vi "Advanced SCP File Download.vi"() -> ()   [LabVIEW 2018]
doc: "Downloads, or receives, any file from a remote SSH server in an efficient, iterative manner. This is similar to the SCP command line utility when transferring, or copying, a remote file to a local destination. Provides advanced functionality to monitoring and optimize performance."
uses:
  Toolkit/Session/Support/Create from SSH.vi
  Toolkit/Session/Support/Password Authentication.vi
  Toolkit/Channel/Support/Create from SCP Receive.vi
  Toolkit/Channel/Support/Destroy to Session.vi
  Toolkit/Session/Support/Destroy to SSH.vi
  Toolkit/SSH/SSH.lvclass
  Toolkit/Session/Session.lvclass
  Toolkit/Channel/Channel.lvclass
panel:
  in  "Abort Download":bool
  out "Download Progress":dbl(slide) scale=0.0..1.0
  out "Bytes Downloaded":u64
  out "Block Download Rate":dbl format="%.3p"
  out "File Download Rate":dbl format="%.3p"
  out "File Download Time":dbl format="%<%H:%M:%S%3u>t"
  in  "Block Size":u64=30000 max=30000
  in  "Remote File":string
  in  "Local File":path
  in  "Remote SSH Server":string
  in  "Password":string
  in  "Username":string
  # "Overview: Demonstrates transferring, or downloading, a remote file from a SSH server, similar to the SCP command line utility with advanced functionality\nInstructions:\n1. Enter the IP address or host name of the remote SSH server. This can be a CompactRIO (cRIO) running the National Instruments Linux Real-Time (NI Linux RT) operating system with the Enable Secure Shell Server (sshd) checkbox checked. \n2. Enter a username. If using a cRIO with a default configuration, then the username is \"admin\".\n3. Enter a password for the username. If using a cRIO with a default configuration, then the password is blank (empty).\n4. Enter the path and/or filename of the remote file to download. Typically, this is a POSIX/UNIX file path with a backslash, \"/\", use to separate directories and the default directory is the remote user's home directory, i.e. \"/home/admin\" on a default configured cRIO.\n5. Select a destination on the local computer for the transfer/download from the remote SSH server.\n6. Run this VI."
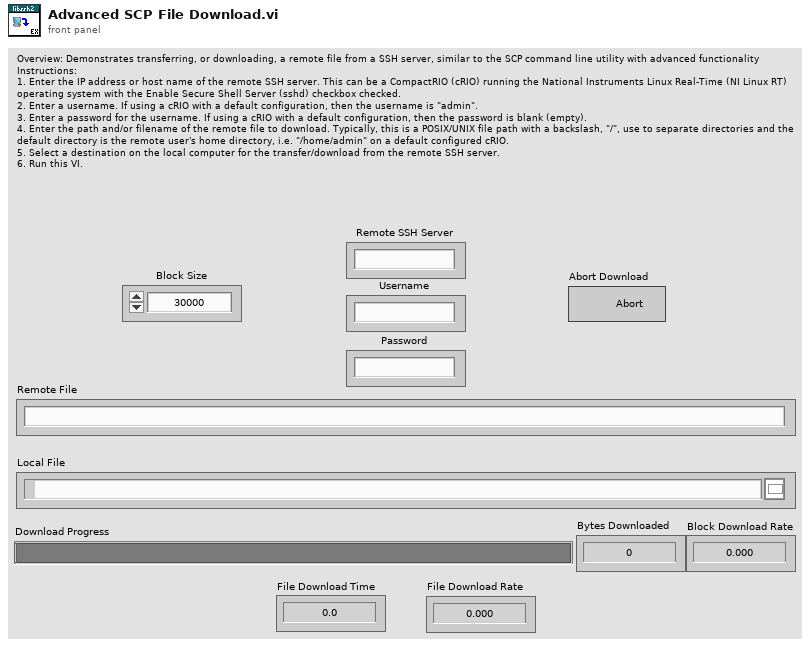
[diagram p1: front panel]
types:
  T1 = enum16{"open", "replace", "create", "open or create", "replace or create", "replace or create with confirmation"}
  T2 = typedef "Toolkit.lvlib/Permissions.ctl" = cluster{"Owner":T3, "Group":T3, "Others":T3}
  T3 = typedef "Toolkit.lvlib/Modes.ctl" = cluster{"Read":bool, "Write":bool, "Execute":bool}
  T4 = cluster{"Access Time":u64, "File Size":u64, "Modified Time":u64, "Permissions":T2}
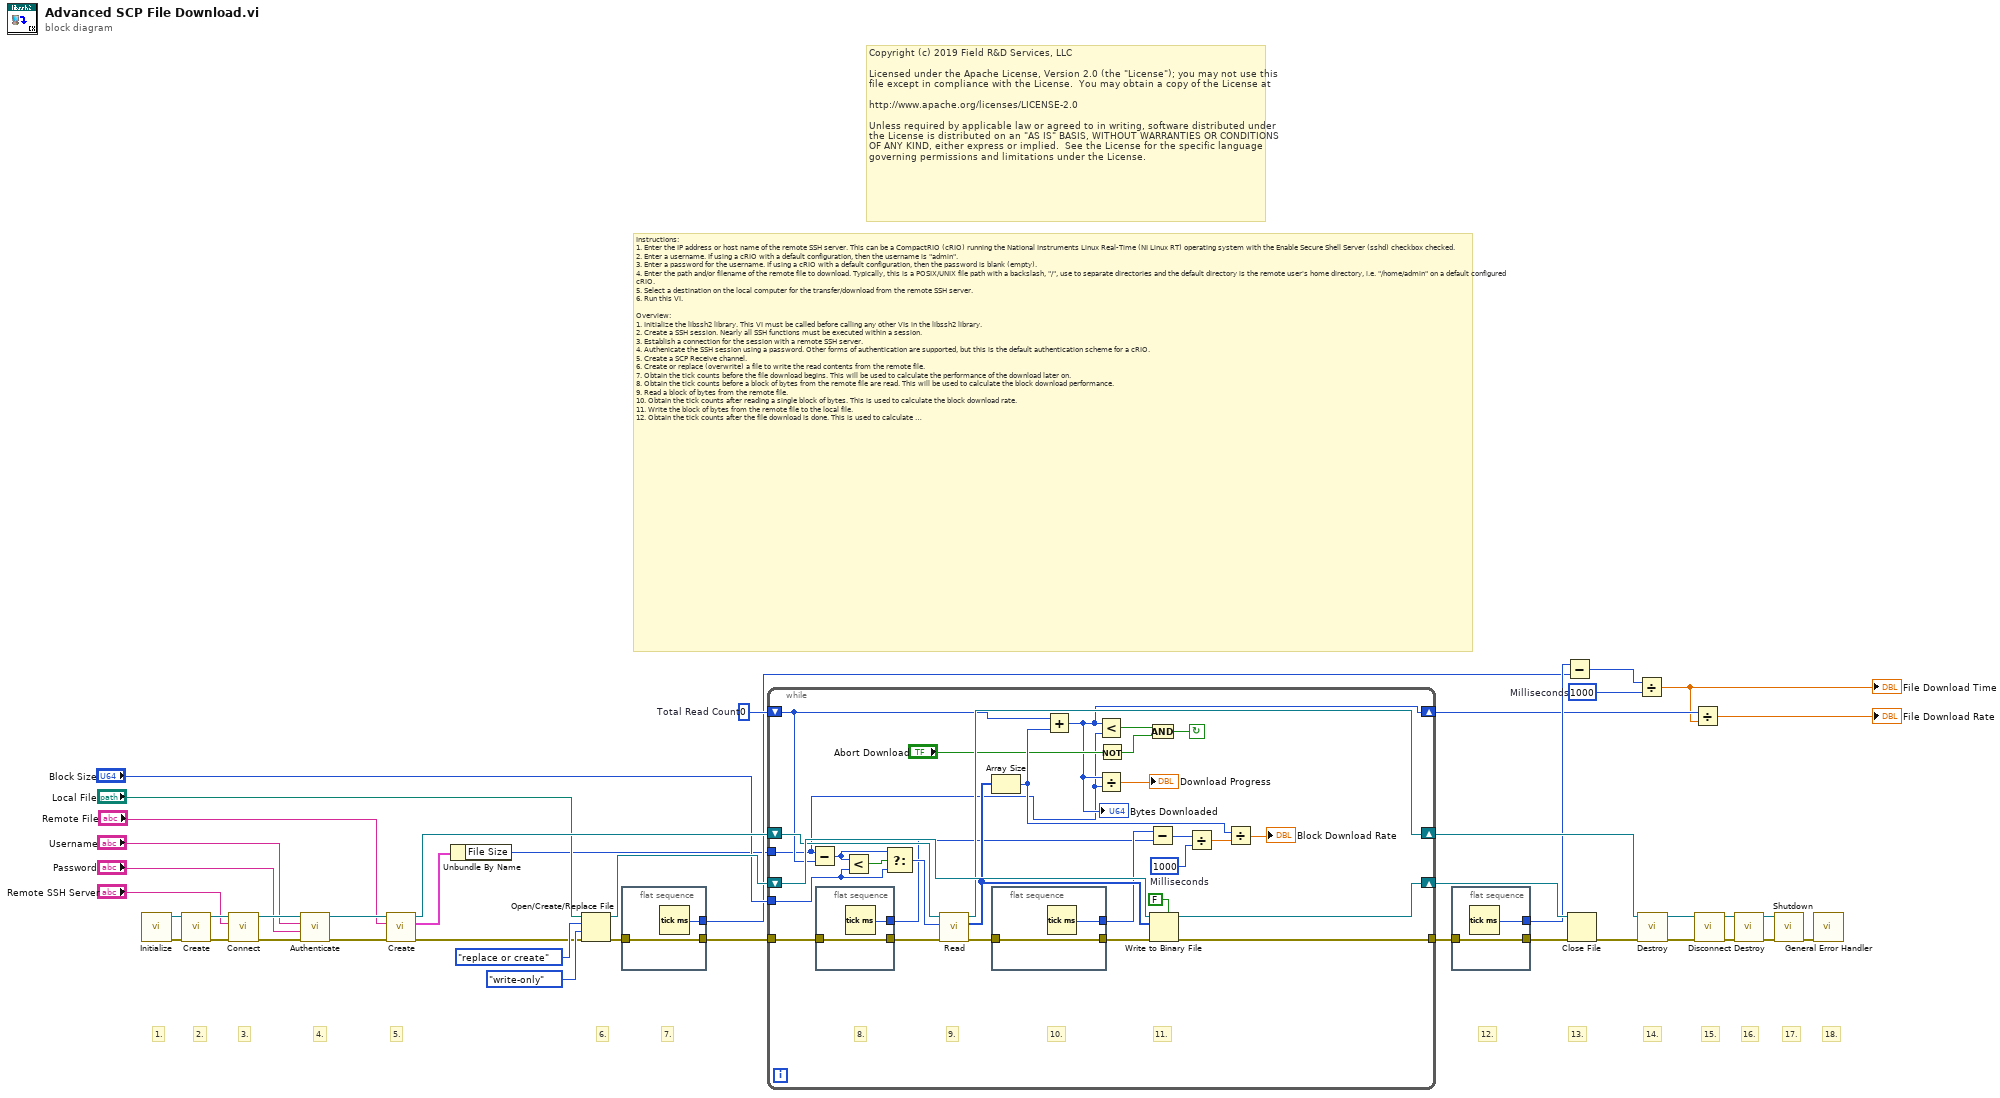
[diagram p0: block diagram]
diagram:
  w10 = u32 1000  # Milliseconds
  w19 = u64 0  # Total Read Count
  # "Copyright (c) 2019 Field R&D Services, LLC\n\nLicensed under the Apache License, Version 2.0 (the \"License\"); you may not use this file except in compliance with the License.  You may obtain a copy of the License at\n\nhttp://www.apache.org/licenses/LICENSE-2.0\n\nUnless required by applicable law or agreed to in writing, software distributed under the License is distributed on an \"AS IS\" BASIS, WITHOUT WARRANTIES OR CONDITIONS OF ANY KIND, either express or implied.  See the License for the specific language governing permissions and limitations under the License."
  # "14."
  # "13."
  # "12."
  # "18."
  # "17."
  # "16."
  # "15."
  # "7."
  # "6."
  # "5."
  # "4."
  # "3."
  # "2."
  # "1."
  # "Instructions:\n1. Enter the IP address or host name of the remote SSH server. This can be a CompactRIO (cRIO) running the National Instruments Linux Real-Time (NI Linux RT) operating system with the Enable Secure Shell Server (sshd) checkbox checked. \n2. Enter a username. If using a cRIO with a default configuration, then the username is \"admin\".\n3. Enter a password for the username. If using a cRIO with a default configuration, then the password is blank (empty).\n4. Enter the path and/or filename of the remote file to download. Typically, this is a POSIX/UNIX file path with a backslash, \"/\", use to separate directories and the default directory is the remote user's home directory, i.e. \"/home/admin\" on a default configured cRIO.\n5. Select a destination on the local computer for the transfer/download from the remote SSH server.\n6. Run this VI.\n\nOverview:\n1. Initialize the libssh2 library. This VI must be called before calling any other VIs in the libssh2 library.\n2. Create a SSH session. Nearly all SSH functions must be executed within a session.\n3. Establish a connection for the session with a remote SSH server.\n4. Authenicate the SSH session using a password. Other forms of authentication are supported, but this is the default authentication scheme for a cRIO. \n5. Create a SCP Receive channel.\n6. Create or replace (overwrite) a file to write the read contents from the remote file.\n7. Obtain the tick counts before the file download begins. This will be used to calculate the performance of the download later on.\n8. Obtain the tick counts before a block of bytes from the remote file are read. This will be used to calculate the block download performance.\n9. Read a block of bytes from the remote file.\n10. Obtain the tick counts after reading a single block of bytes. This is used to calculate the block download rate.\n11. Write the block of bytes from the remote file to the local file.\n12. Obtain the tick counts after the file download is done. This is used to calculate the file download time and rate.\n13. Close the file. This is not strictly necessary, but it is good practice.\n14. Destroy the SCP Receive channel. Since the \"Create\" VI is used, the complementary \"Destroy\" VI must be used to free resources within the libssh2 library.\n15. Disconnect from the remote SSH server.\n16. Destroy the session to free resources within the libssh2 library.\n17. Shutdown the libssh2 library. This VI must be last VI called for the libssh2 library. No other libssh2 VIs should be called once this VI is executed.\n18. Provide some error handling and reporting. Libssh2 errors will be in the -8100 range."
  n1 = call "Initialize.vi"() -> ("Error Out"=w30:errorcluster, "SSH"=w29:refnum<class "SSH.lvclass">)  [unwired: 10 in]
  n2 = call-poly "Create.vi"("Error In"=w30, "SSH"=w29) -> ("Error Out"=w42:errorcluster, "Sesssion"=w43:refnum<class "Session.lvclass">)  [unwired: 8 in]
  n3 = call "Connect.vi"("Error In"=w42, "Address"="Remote SSH Server", "Session In"=w43) -> ("Error Out"=w40:errorcluster, "Sesssion Out"=w41:refnum<class "Session.lvclass">)  [unwired: 7 in]
  n4 = call-poly "Authenticate.vi"("Error In"=w40, "Password"="Password", "Username"="Username", "Session In"=w41) -> ("Error Out"=w5:errorcluster, "Sesssion Out"=w6:refnum<class "Session.lvclass">)  [unwired: 6 in]
  n5 = call-poly "Create.vi"("Error In"=w5, "Remote Source Path"="Remote File", "Session"=w6) -> ("Error Out"=w4:errorcluster, "File Information"=w2:T4, "Channel"=w28:refnum<class "Channel.lvclass">)  [unwired: 6 in]
  n6 = Unbundle By Name(w2) -> ("File Size"=w1:u64)
  n7 = Open/Create/Replace File(file path (use dialog)="Local File", error in=w4, operation (0:open)=T1."replace or create", access (0:read/write)=enum16{"read/write", "read-only", "write-only"}."write-only") -> (refnum out=w24:refnum<file>, error out=w17:errorcluster)  [unwired: 2 in, 1 out]
  n8 = flat-sequence {
    tunnel: w17 -> [w45]
    tunnel: [w45] -> w16
    tunnel: [w44] -> w12
    frame #0 {
      n9 = Tick Count (ms)() -> (millisecond timer value=w44:u32)
    }
  }
  n10 = while {
    shift-right: [w75] -> w22
    shift-left: w24 -> [w73]
    tunnel: w16 -> [w64]
    shift-right: [w71] -> w23
    shift-left: w28 -> [w72]
    tunnel: [w74] -> w15
    shift-right: [w49] -> w9
    shift-left: w19 -> [w68]
    tunnel: w1 -> [w48]
    tunnel: "Block Size" -> [w65]
    stop <- w51 continue-if-true
    w57 = u32 1000  # Milliseconds
    # "10."
    # "9."
    # "8."
    # "11."
    n11 = Subtract(x=w48, y=w68) -> (x-y=w67:u64)
    n12 = flat-sequence {
      tunnel: w64 -> [w79]
      tunnel: [w79] -> w63
      tunnel: [w78] -> w59
      frame #0 {
        n13 = Tick Count (ms)() -> (millisecond timer value=w78:u32)
      }
    }
    n14 = Less?(x=w67, y=w65) -> (x < y?=w69:bool)
    n15 = Select(t=w67, s=w69, f=w65) -> (s? t:f=w66:u64)
    n16 = call "Read.vi"("Error In"=w63, "Max Data Length"=w66, "Channel In"=w72) -> ("Error Out"=w62:errorcluster, "Data"=w70:u8[], "Channel Out"=w71:refnum<class "Channel.lvclass">)  [unwired: 6 in]
    n17 = Array Size(array=w70) -> (size(s)=w55:i32)
    n18 = flat-sequence {
      tunnel: w62 -> [w77]
      tunnel: [w77] -> w61
      tunnel: [w76] -> w60
      frame #0 {
        n19 = Tick Count (ms)() -> (millisecond timer value=w76:u32)
      }
    }
    n20 = Add(x=w68, y=w55) -> (x+y=w49:u64)
    "Bytes Downloaded" <- w49
    n21 = Less?(x=w49, y=w48) -> (x < y?=w52:bool)
    n22 = Divide(x=w49, y=w48) -> (x/y=→"Download Progress":dbl)
    n23 = Not(x="Abort Download") -> (.not. x?=w50:bool)
    n24 = Subtract(x=w60, y=w59) -> (x-y=w58:u32)
    n25 = And(x=w52, y=w50) -> (x .and. y?=w51:bool)
    n26 = Write to Binary File(file (use dialog)=w73, data=w70, error in=w61, 5:FALSE ("prepend array or string size? (T)")) -> (refnum out=w75:refnum<file>, error out=w74:errorcluster)  [unwired: 2 in, 1 out]
    n27 = Divide(x=w58, y=w57) -> (x/y=w56:dbl)
    n28 = Divide(x=w55, y=w56) -> (x/y=→"Block Download Rate":dbl)
  }
  n29 = flat-sequence {
    tunnel: w15 -> [w81]
    tunnel: [w81] -> w14
    tunnel: [w80] -> w13
    frame #0 {
      n30 = Tick Count (ms)() -> (millisecond timer value=w80:u32)
    }
  }
  n31 = Subtract(x=w13, y=w12) -> (x-y=w11:u32)
  n32 = Close File(refnum=w22, error in=w14) -> (error out=w21:errorcluster)  [unwired: 1 out]
  n33 = Divide(x=w11, y=w10) -> (x/y=w8:dbl)
  "File Download Time" <- w8
  n34 = call-poly "Destroy.vi"("Error In"=w21, "Channel"=w23) -> ("Error Out"=w35:errorcluster, "Session"=w36:refnum<class "Session.lvclass">)  [unwired: 8 in]
  n35 = Divide(x=w9, y=w8) -> (x/y=→"File Download Rate":dbl)
  n36 = call "Disconnect.vi"("Error In"=w35, "Session In"=w36) -> ("Error Out"=w33:errorcluster, "Sesssion Out"=w34:refnum<class "Session.lvclass">)  [unwired: 8 in]
  n37 = call-poly "Destroy.vi"("Error In"=w33, "Session"=w34) -> ("Error Out"=w31:errorcluster, "SSH"=w32:refnum<class "SSH.lvclass">)  [unwired: 8 in]
  n38 = call "Shutdown.vi"("Error In"=w31, "SSH"=w32) -> ("Error Out"=w20:errorcluster)  [unwired: 9 in]
  n39 = call <vilib>:"General Error Handler.vi"("error in (no error)"=w20) -> ()  [unwired: 10 in, 5 out]
